vi "Read Day Entries.vi"(8 "error in (no error)":errorcluster, 10 "Date":timestamp, 11 "Data Folder":path) -> (0 "error out":errorcluster, 3 "Time Entries":T1)   [LabVIEW 2024]
doc: "Returns the time entries whose Start Time falls on the given LOCAL calendar day (midnight to midnight in the time zone of the computer), sorted by Start Time. Because month files are bucketed by UTC, a local day can span two files; both are read when it does. The day is taken as 24 hours from local midnight.\n\nGenerated by: Claude"
uses:
  Rows/Time Entry.ctl
  Rows/Time Entry List.ctl
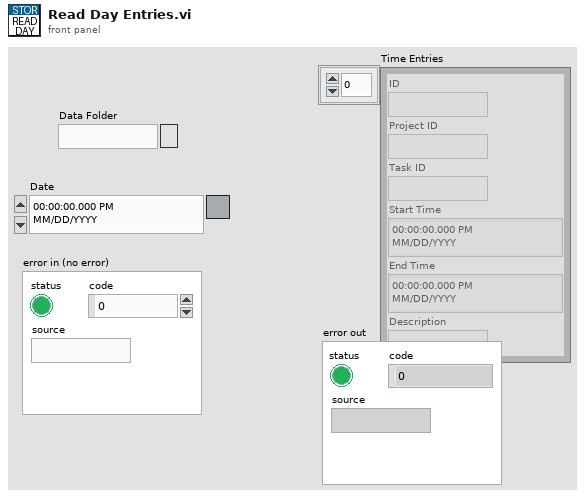
[diagram p1: front panel]
types:
  T1 = typedef "Time Entry List.ctl" = T2[]
  T2 = typedef "Time Entry.ctl" = cluster{"ID":string, "Project ID":string, "Task ID":string, "Start Time":timestamp, "End Time":timestamp, "Description":string}
  T3 = typedef "LVDateTimeRec.ctl" = cluster{"fractional second":dbl, "second":i32, "minute":i32, "hour":i32, "day of month":i32, "month":i32, "year":i32, "day of week":i32, "day of year":i32, "DST":i32}
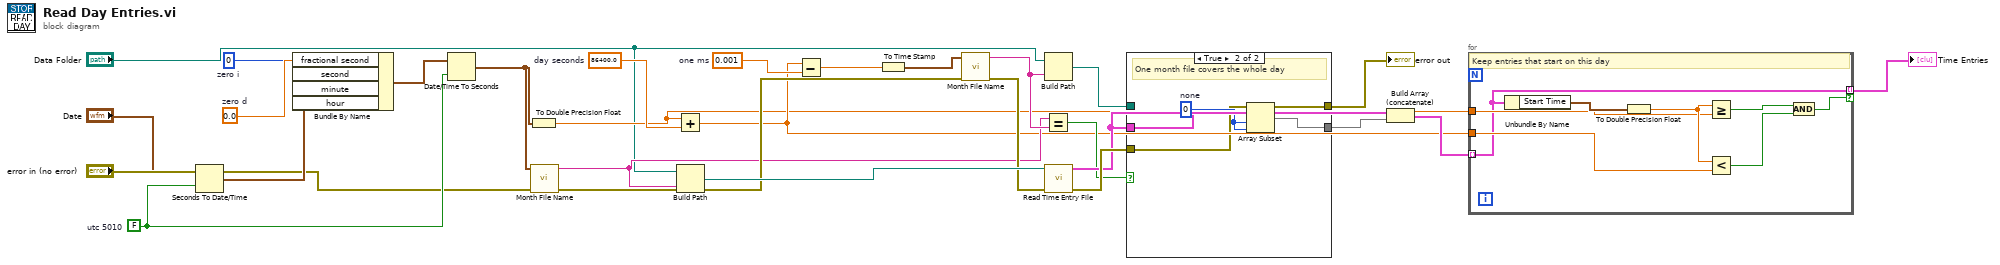
[diagram p0: block diagram]
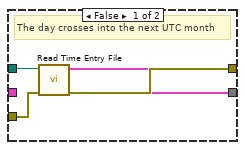
[diagram p2: hidden frame]
diagram:
  w13 = 0.001  # one ms
  w11 = 86400.0  # day seconds
  w6 = FALSE  # utc 5010
  w5 = 0.0  # zero d
  w4 = 0  # zero i
  n1 = Seconds To Date/Time(time stamp (now)="Date", to UTC (F)=w6) -> (date time rec=w7:T3)
  n2 = Bundle By Name(cluster=w7, "fractional second"=w5, "second"=w4, "minute"=w4, "hour"=w4) -> (w8:T3)
  n3 = Date/Time To Seconds(1:w6, 2:w8) -> (0:w9:timestamp)
  n4 = To Double Precision Float(number=w9) -> (double precision float=w10:dbl)
  n5 = call "Month File Name.vi"("error in (no error)"="error in (no error)", "Start Time"=w9) -> ("error out"=w17:errorcluster, "File Name"=w16:string)  [unwired: 8 in]
  n6 = Add(x=w10, y=w11) -> (x+y=w12:dbl)
  n7 = Build Path(base path="Data Folder", name or relative path=w16) -> (appended path=w20:path)
  n8 = Subtract(x=w12, y=w13) -> (x-y=w14:dbl)
  n9 = To Time Stamp(1:w14) -> (0:w15:timestamp)
  n10 = call "Month File Name.vi"("error in (no error)"=w17, "Start Time"=w15) -> ("error out"=w19:errorcluster, "File Name"=w18:string)  [unwired: 8 in]
  n11 = Build Path(base path="Data Folder", name or relative path=w18) -> (appended path=w21:path)
  n12 = Equal?(x=w16, y=w18) -> (x = y?=w22:bool)
  n13 = call "Read Time Entry File.vi"("error in (no error)"=w19, "File Path"=w20) -> ("error out"=w24:errorcluster, "Time Entries"=w23:T1)  [unwired: 6 in, 2 out]
  n14 = case shown="True" w22 {
    tunnel: w21 -> [w29 _]
    tunnel: w23 -> [_ w33]
    tunnel: w24 -> [w30 w34]
    tunnel: [w32 w34] -> w26
    tunnel: [w31 w36] -> w25
    frame False {
      # "The day crosses into the next UTC month"
      n15 = call "Read Time Entry File.vi"("error in (no error)"=w30, "File Path"=w29) -> ("error out"=w32:errorcluster, "Time Entries"=w31:T1)  [unwired: 6 in, 2 out]
    }
    frame True {
      w35 = 0  # none
      # "One month file covers the whole day"
      n16 = Array Subset(array=w33, index=w35, length=w35) -> (w36:T1)
    }
  }
  "error out" <- w26
  n17 = Build Array (concatenate)(w23, w25) -> (w27:T1)
  n18 = for {
    tunnel: w10 -> [w38]
    tunnel: w12 -> [w39]
    tunnel: w27 -> [w37] mode=indexing
    tunnel: [w37] -> w28 mode=indexing if=w44
    # "Keep entries that start on this day"
    n19 = Unbundle By Name(w37) -> ("Start Time"=w40:timestamp)
    n20 = To Double Precision Float(number=w40) -> (double precision float=w41:dbl)
    n21 = Greater Or Equal?(x=w41, y=w38) -> (x >= y?=w42:bool)
    n22 = Less?(x=w41, y=w39) -> (x < y?=w43:bool)
    n23 = And(x=w42, y=w43) -> (x .and. y?=w44:bool)
  }
  "Time Entries" <- w28
